vi "D_W_SD_Array.vi"(8 "error in (no error)":errorcluster, 9 "slotNo":u32, 10 "2D array":u8[][](array[numeric]), 11 "bID":u8) -> (0 "error out":errorcluster, 3 "bID":u8, 4 "TorF":i32)   [LabVIEW 2017]
uses:
  LabVIEW2018/hpkSLMdaLV.dll
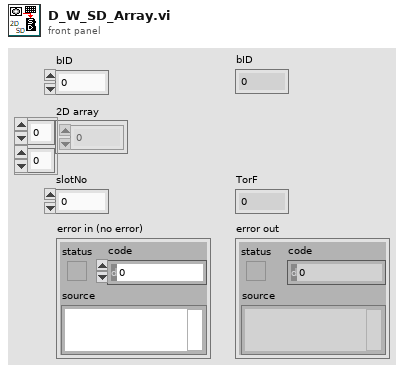
[diagram p1: front panel]
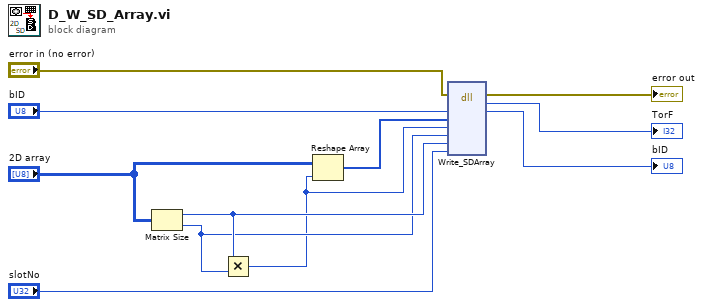
[diagram p0: block diagram]
diagram:
  n1 = Matrix Size(0:"2D array") -> (1:w11:i32, 2:w10:i32)
  n2 = Multiply(x=w11, y=w10) -> (x*y=w9:i32)
  n3 = Reshape Array("2D array", w9) -> (w8:u8[])
  n4 = dll-call lib="C:/Users/hs5921/Desktop/LabVIEW2018/hpkSLMdaLV.dll" fn="Write_SDArray"(error in="error in (no error)", "bID"="bID", "arrayIn"=w8, "arraySize"=w9, "XPixel"=w10, "YPixel"=w11, "SDSlotNo"="slotNo") -> (error out=→"error out":errorcluster, "返り値タイプ"=→"TorF":i32, "bID"=→"bID":u8)  [unwired: 7 in, 1 out]
